vi "register-reflection-descriptors.old.vi"(8 "error in":errorcluster, 11 "reflector description strings":string[](array[string])) -> (0 "error out":errorcluster)   [LabVIEW 2019, in "grpc-lvsupport.lvlib"]
uses:
  grpc-lvsupport.lvlib
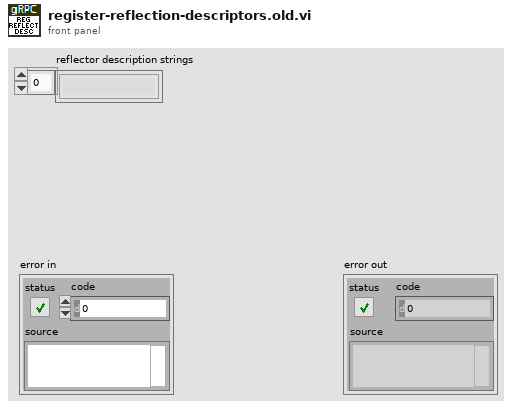
[diagram p1: front panel]
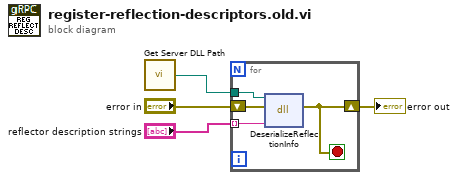
[diagram p0: block diagram]
diagram:
  n1 = call "Get Server DLL Path.vi"() -> ("server dll path"=w3:path)
  n2 = for {
    tunnel: w3 -> [w8]
    tunnel: "reflector description strings" -> [w7] mode=indexing
    shift-right: [w5] -> w4
    shift-left: "error in" -> [w6]
    stop <- w5 stop-if-true
    n3 = dll-call lib="?" fn="DeserializeReflectionInfo"(path in=w8, error in=w6, "serializedDescriptor"=w7) -> (error out=w5:errorcluster)  [unwired: 3 in, 1 out]
  }
  "error out" <- w4
